vi "Test Open Close.vi"() -> ()   [LabVIEW 2021]
uses:
  CAN RW CANsub.lvclass
  <vilib>/CIF Foundation/CIF CAN RW Core/typedef/CAN Mode.ctl
  <vilib>/CIF Foundation/CIF CAN RW Core/CAN_RW_CORE.lvclass
  <vilib>/CIF Foundation/CIF CAN RW Core/typedef/FD Config.ctl
  <vilib>/CIF Foundation/CIF CAN RW Core/typedef/CAN Port Configuration.ctl
panel:
  out "error out":errorcluster
  in  "open time ms":u32=5000
  in  "writer":bool
  in  "Port Configuration":T1={"Mode"=enum."CAN FD", "Baud Rate"=500000, "Temination On"=TRUE, "Subordinate"=FALSE, "Echo TX"=FALSE, "FD Config"={"FD Baud Rate"=2000000, "ISO Mode"=TRUE, "BRS Enabled"=TRUE}} {"FD Config"."FD Baud Rate" format="%.0p"; "Baud Rate" format="%.0p"}
  in  "Interface":string="192.168.0.49/2"
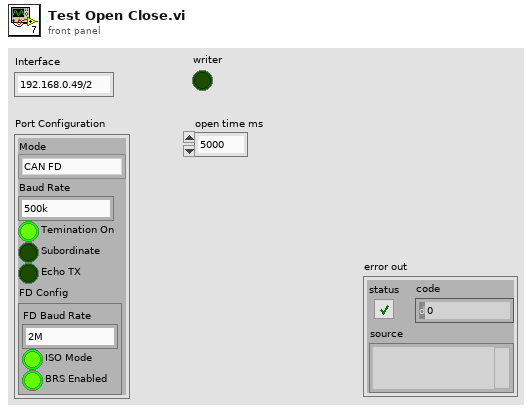
[diagram p1: front panel]
types:
  T1 = typedef "CAN_RW_CORE.lvclass/CAN Port Configuration.ctl" = cluster{"Mode":T2, "Baud Rate":u64, "Temination On":bool, "Subordinate":bool, "Echo TX":bool, "FD Config":T3}
  T2 = typedef "CAN_RW_CORE.lvclass/CAN Mode.ctl" = enum16{"CAN 2.0", "CAN FD"}
  T3 = typedef "CAN_RW_CORE.lvclass/FD Config.ctl" = cluster{"FD Baud Rate":u64, "ISO Mode":bool, "BRS Enabled":bool}
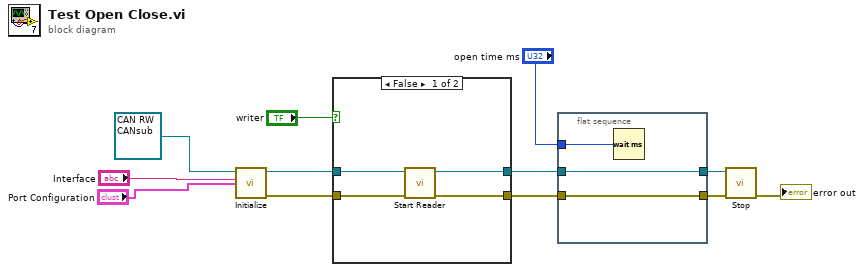
[diagram p0: block diagram]
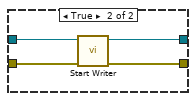
[diagram p2: hidden frame]
diagram:
  n1 = call "Initialize.vi"("Port Configuration"="Port Configuration", "Interface"="Interface", "CANsub_CAN_RW in"=refnum<class "CAN RW CANsub.lvclass"> refnum ("CAN RW CANsub.lvclass")) -> ("error out"=w7:errorcluster, "CANsub_CAN_RW out"=w8:refnum<class "CAN RW CANsub.lvclass">)  [unwired: 7 in]
  n2 = case shown="False" "writer" {
    tunnel: w8 -> [w16 w20]
    tunnel: [w15 w19] -> w5
    tunnel: w7 -> [w14 w18]
    tunnel: [w13 w17] -> w4
    frame False {
      n3 = call-dynamic "Start Reader.vi"("error in (no error)"=w14, "CAN RW CANsub in"=w16) -> ("error out"=w13:errorcluster, "CAN RW CANsub out"=w15:refnum<class "CAN RW CANsub.lvclass">)  [unwired: 8 in]
    }
    frame True {
      n4 = call-dynamic "Start Writer.vi"("error in (no error)"=w18, "CAN RW CANsub in"=w20) -> ("error out"=w17:errorcluster, "CAN RW CANsub out"=w19:refnum<class "CAN RW CANsub.lvclass">)  [unwired: 8 in]
    }
  }
  n5 = flat-sequence {
    tunnel: "open time ms" -> [w23]
    tunnel: [w22] -> w3
    tunnel: w5 -> [w22]
    tunnel: [w21] -> w2
    tunnel: w4 -> [w21]
    frame #0 {
      n6 = Wait (ms)(milliseconds to wait=w23) -> ()  [unwired: 1 out]
    }
  }
  n7 = call-dynamic "Stop.vi"("error in (no error)"=w2, "CAN RW CANsub in"=w3) -> ("error out"=→"error out":errorcluster)  [unwired: 8 in, 1 out]
